vi "Tell Reply.vi"(4 "Priority":bool, 7 "Actor in":refnum<class "Actor.lvclass">, 8 "Error in":errorcluster, 10 "Msg":refnum<class "Msg.lvclass">) -> (0 "Error out":errorcluster, 5 "Actor out":refnum<class "Actor.lvclass">)   [LabVIEW 2020, in "jettl.lvlib"]
uses:
  jettl.lvlib
  Msg/Msg.lvclass
  Actor/Actor.lvclass
  Teller/Teller.lvclass
  Msg Input/Msg Input.lvclass
  Attributes/Attributes.lvclass
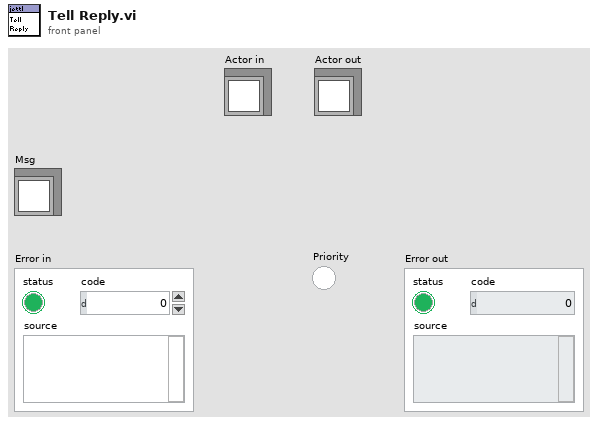
[diagram p1: front panel]
types:
  T1 = typedef "jettl.lvlib/Relation.ctl" = enum16{"Self", "Parent", "Child", "No Relation"}
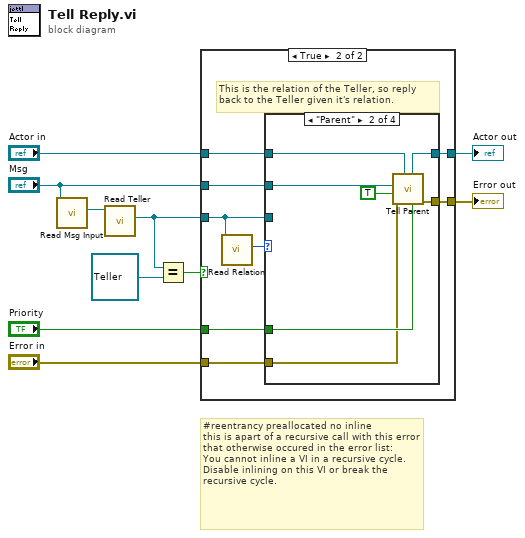
[diagram p0: block diagram]
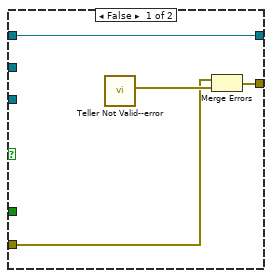
[diagram p2: hidden frame]
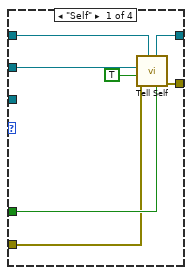
[diagram p3: hidden frame]
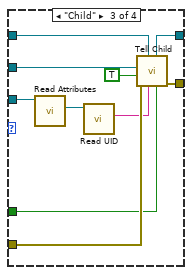
[diagram p4: hidden frame]
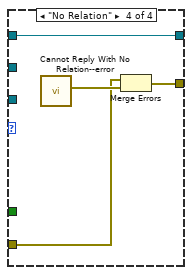
[diagram p5: hidden frame]
diagram:
  # "#reentrancy preallocated no inline\nthis is apart of a recursive call with this error that otherwise occured in the error list:\nYou cannot inline a VI in a recursive cycle. Disable inlining on this VI or break the recursive cycle."
  n1 = call-dynamic "Read Msg Input.vi"("Msg in"="Msg") -> ("Msg Input"=w5:refnum<class "Msg Input.lvclass">)  [unwired: 10 in]
  n2 = call-dynamic "Read Teller.vi"("Msg Input in"=w5) -> ("Teller"=w3:refnum<class "Teller.lvclass">)  [unwired: 10 in]
  n3 = Equal?(x=w3, y=refnum<class "Teller.lvclass"> refnum ("Sender")) -> (x = y?=w8:bool)
  n4 = case shown="True" w8 {
    tunnel: "Actor in" -> [w13 w22]
    tunnel: "Msg" -> [_ w21]
    tunnel: "Priority" -> [_ w20]
    tunnel: w3 -> [_ w19]
    tunnel: [w12 w17] -> w9
    tunnel: [w13 w16] -> w2
    tunnel: "Error in" -> [w11 w15]
    frame False {
      n5 = call "Teller Not Valid--error.vi"() -> ("Error"=w14:errorcluster)  [unwired: 11 in]
      n6 = Merge Errors(w11, w14) -> (w12:errorcluster)
    }
    frame True {
      # "This is the relation of the Teller, so reply back to the Teller given it's relation."
      n7 = call-dynamic "Read Relation.vi"("Teller in"=w19) -> ("Relation"=w18:T1)  [unwired: 10 in]
      n8 = case shown="\"Parent\"" w18 {
        tunnel: w22 -> [w29 w36 w44 w49]
        tunnel: w21 -> [w28 w35 w43 _]
        tunnel: w20 -> [w27 w34 w38 _]
        tunnel: w19 -> [_ _ w46 _]
        tunnel: [w26 w33 w42 w48] -> w17
        tunnel: [w25 w31 w41 w49] -> w16
        tunnel: w15 -> [w24 w32 w40 w47]
        frame "Self" {
          n9 = call "Tell Self.vi"("Priority"=w27, "Actor in"=w29, "Error in"=w24, "Reply"=TRUE, "Msg"=w28) -> ("Error out"=w26:errorcluster, "Actor out"=w25:refnum<class "Actor.lvclass">)  [unwired: 5 in]
        }
        frame "Parent" {
          n10 = call "Tell Parent.vi"("Priority"=w34, "Actor in"=w36, "Error in"=w32, "Reply"=TRUE, "Msg"=w35) -> ("Error out"=w33:errorcluster, "Actor out"=w31:refnum<class "Actor.lvclass">)  [unwired: 5 in]
        }
        frame "Child" {
          n11 = call-dynamic "Read Attributes.vi"("Teller in"=w46) -> ("Attributes"=w45:refnum<class "Attributes.lvclass">)  [unwired: 10 in]
          n12 = call-dynamic "Read UID.vi"("Attributes in"=w45) -> ("UID"=w39:string)  [unwired: 10 in]
          n13 = call "Tell Child.vi"("Priority"=w38, "UID"=w39, "Actor in"=w44, "Error in"=w40, "Reply"=TRUE, "Msg"=w43) -> ("Error out"=w42:errorcluster, "Actor out"=w41:refnum<class "Actor.lvclass">)  [unwired: 4 in]
        }
        frame "No Relation" {
          n14 = call "Cannot Reply With No Relation--error.vi"() -> ("Error"=w50:errorcluster)  [unwired: 11 in]
          n15 = Merge Errors(w47, w50) -> (w48:errorcluster)
        }
      }
    }
  }
  "Error out" <- w9
  "Actor out" <- w2
